vi "set Y-axis Unit.vi"(8 "error in (no error)":errorcluster, 10 "Y-axis Unit":T1, 11 "Keysight 9020A in":refnum<class "Keysight 9020A.lvclass">) -> (0 "error out":errorcluster, 3 "Keysight 9020A out":refnum<class "Keysight 9020A.lvclass">)   [LabVIEW 2023, in "Spectrum Analyzer.lvlib" / "Keysight 9020A.lvclass"]
uses:
  Keysight 9020A.lvclass
  Keysight 9020A.lvclass/Keysight 9020A.ctl
  TYPE DEFINITION/TYPE Y-axis Unit.ctl
  Spectrum Analyzer.lvlib
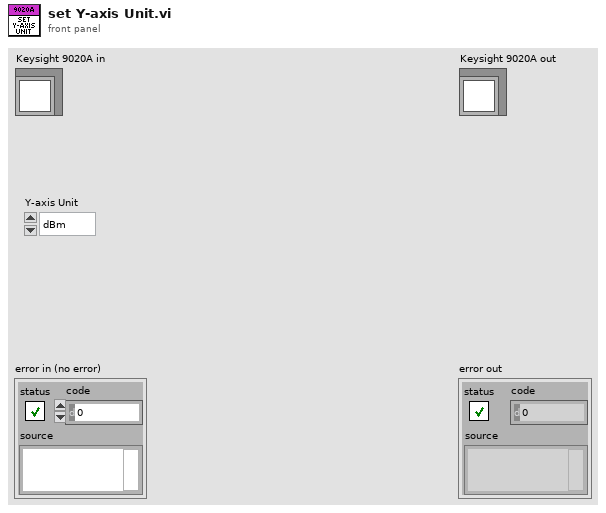
[diagram p1: front panel]
types:
  T1 = typedef "Spectrum Analyzer.lvlib/TYPE Y-axis Unit.ctl" = enum16{"dBm", "dBmV", "dBuV", "dBpW", "Volt", "Ampere", "Watt"}
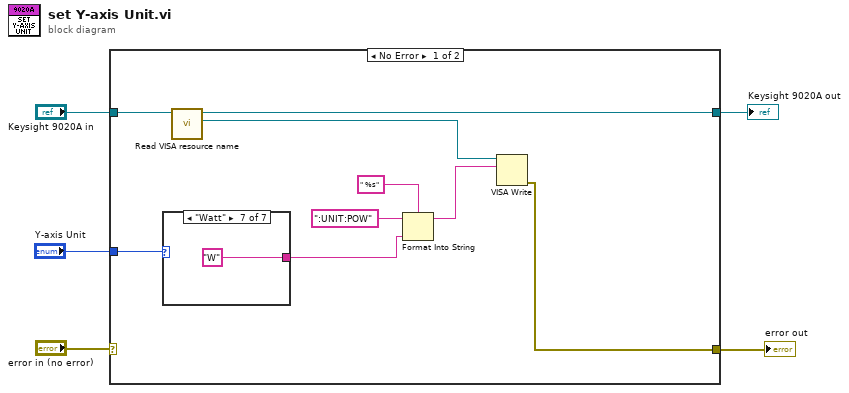
[diagram p0: block diagram]
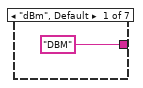
[diagram p2: hidden frame]
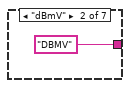
[diagram p3: hidden frame]
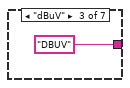
[diagram p4: hidden frame]
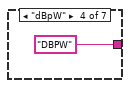
[diagram p5: hidden frame]
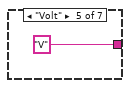
[diagram p6: hidden frame]
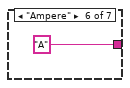
[diagram p7: hidden frame]
diagram:
  n1 = case shown="No Error" "error in (no error)" {
    selector: "error in (no error)" -> [_ w22]
    tunnel: "Keysight 9020A in" -> [w14 w23]
    tunnel: [w13 w23] -> w4
    tunnel: [w6 w22] -> w2
    tunnel: "Y-axis Unit" -> [w12 _]
    frame No Error {
      n2 = case shown="\"Watt\"" w12 {
        tunnel: ["DBM" "DBMV" "DBUV" "DBPW" "V" "A" "W"] -> w9
        frame "dBm", Default {
        }
        frame "dBmV" {
        }
        frame "dBuV" {
        }
        frame "dBpW" {
        }
        frame "Volt" {
        }
        frame "Ampere" {
        }
        frame "Watt" {
        }
      }
      n3 = call "Read VISA resource name.vi"("Keysight 9020A in"=w14) -> ("VISA resource name"=w8:refnum<visa-resource-name>, "Keysight 9020A out"=w13:refnum<class "Keysight 9020A.lvclass">)  [unwired: 8 in, 1 out]
      n4 = Format Into String(format string=" %s", initial string=":UNIT:POW", w9) -> (resulting string=w7:string)  [unwired: 1 in, 1 out]
      n5 = VISA Write(VISA resource name=w8, write buffer=w7) -> (error out=w6:errorcluster)  [unwired: 1 in, 2 out]
    }
    frame Error {
    }
  }
  "error out" <- w2
  "Keysight 9020A out" <- w4
